vi "ASD SearchSpecifedBoolArrayFrom1DBool.vi"(9 "検索する配列":bool[](array[boolean]), 10 "対象とする配列":bool[](array[boolean])) -> (2 "指標":i32)   [LabVIEW 2018]
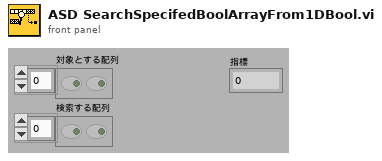
[diagram p1: front panel]
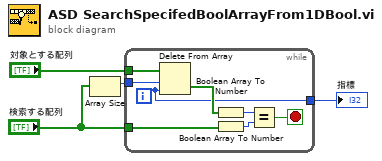
[diagram p0: block diagram]
diagram:
  n1 = Array Size(array="検索する配列") -> (size(s)=w3:i32)
  n2 = while {
    tunnel: "対象とする配列" -> [w12]
    tunnel: w3 -> [w11]
    tunnel: "検索する配列" -> [w9]
    tunnel: [w5] -> w1
    i -> [w5]
    stop <- w6 stop-if-true
    n3 = Delete From Array(array=w12, length=w11, index=w5) -> (deleted portion=w10:bool[])  [unwired: 1 out]
    n4 = Boolean Array To Number(Boolean array=w10) -> (number=w8:u32)
    n5 = Boolean Array To Number(Boolean array=w9) -> (number=w7:u32)
    n6 = Equal?(x=w8, y=w7) -> (x = y?=w6:bool)
  }
  "指標" <- w1
